vi "Variable glob Th.vi"() -> ()   [LabVIEW 2022 SP3]
panel:
  in  "Donnees Th/tache":cluster{"Données Th":string[]}[](array[cluster])
  in  "Taches Th":T1(array[cluster])
  in  "Temp Th":bool
  out "Nb de chassis Th":u8
  # "THERMOCOUPLES"
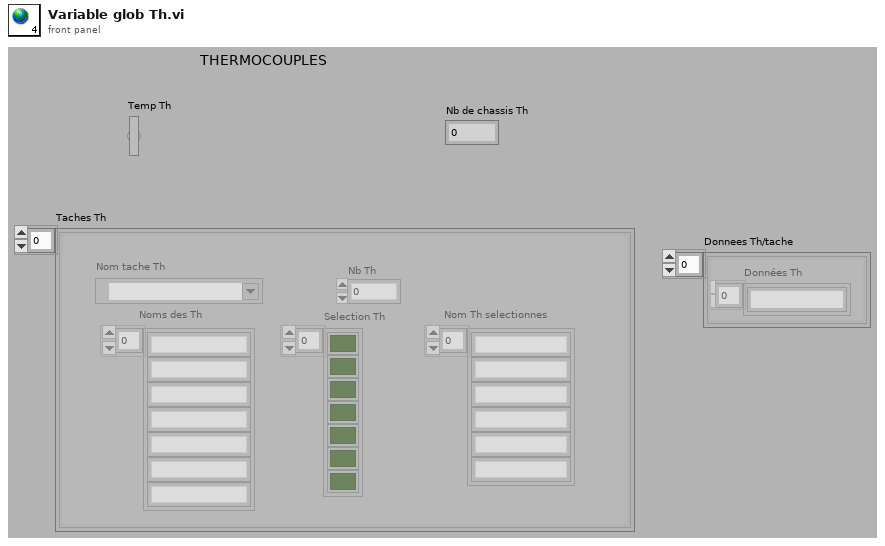
[diagram p1: front panel]
types:
  T1 = cluster{"Nom tache Th":refnum<k21>, "Noms des Th":string[], "Nb Th":i16, "Selection Th":bool[], "Nom Th selectionnes":string[]}[]
diagram:
